vi "Example_Frames_To_Rows.vi"(8 "error in (no error)":errorcluster, 11 "frames":T1 {"flags" format="%.0x"; "id" format="%.0x"}) -> (0 "error out":errorcluster, 3 "rows":string[][](array[string]))   [LabVIEW 2021]
doc: "Example: formats the frames of one Read as table rows (time UTC s, ID hex, flags X/F/B/R/A/E, DLC, data hex) using Frame_Get. Allocates strings; for display only, not for a time-critical loop."
uses:
  api/CANsub_Channel/CANsub_Channel.lvclass
  <vilib>/JDP Science/JDP Science Common Utilities/JDP Utility.lvlib
  api/Typedefs/CANsub_Frames.ctl
  api/CANsub_API.lvlib
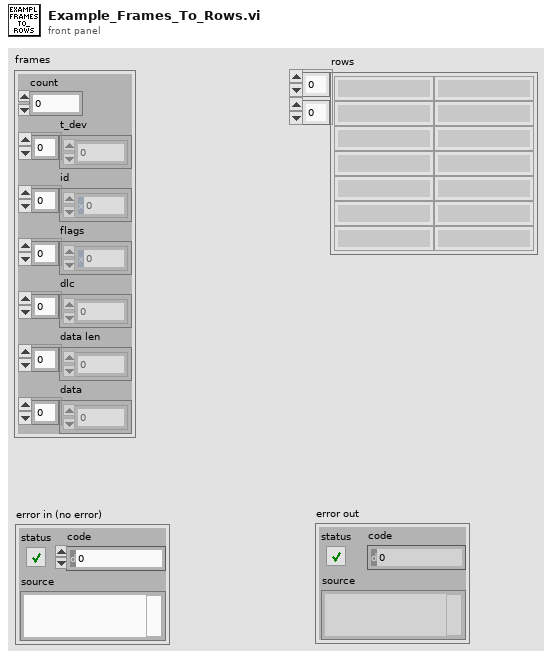
[diagram p1: front panel]
types:
  T1 = typedef "CANsub_API.lvlib/CANsub_Frames.ctl" = cluster{"count":i32, "t_dev":dbl[], "id":u32[], "flags":u16[], "dlc":u8[], "data len":u8[], "data":u8[]}
  T2 = typedef "CANsub_API.lvlib/CANsub_Frame.ctl" = cluster{"id":u32, "t_dev":dbl, "dlc":u8, "data len":u8, "ide":bool, "fdf":bool, "rtr":bool, "brs":bool, "esi":bool, "tx ack":bool, "error frame":bool}
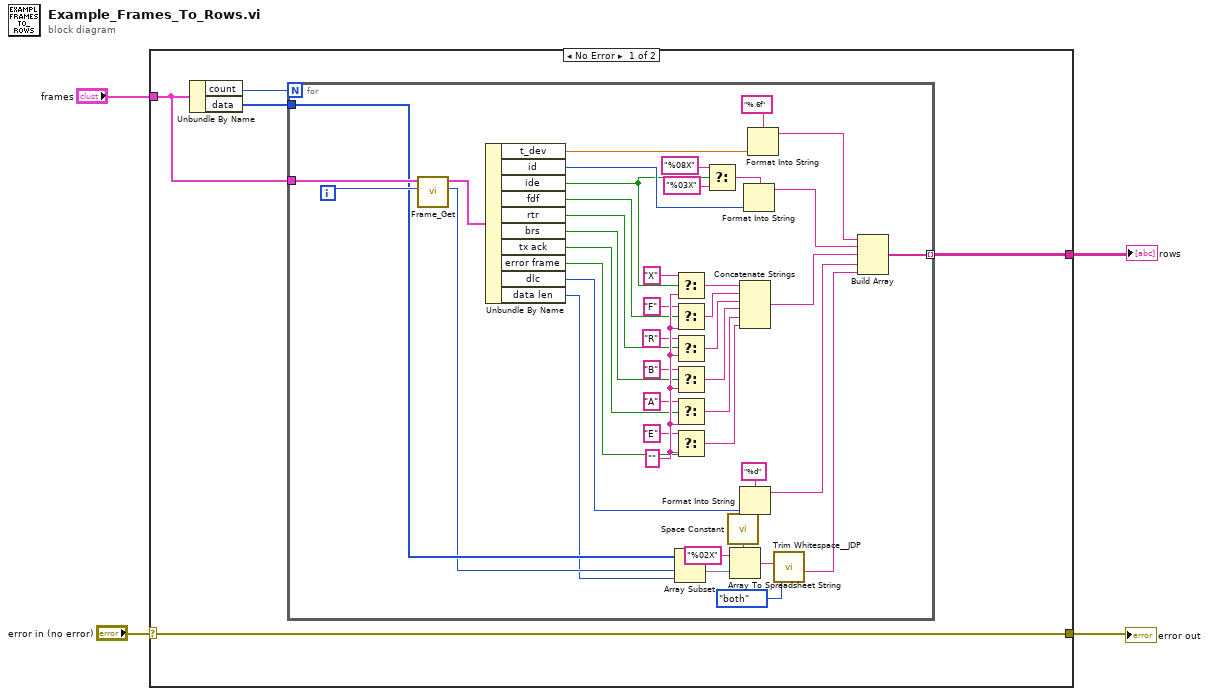
[diagram p0: block diagram]
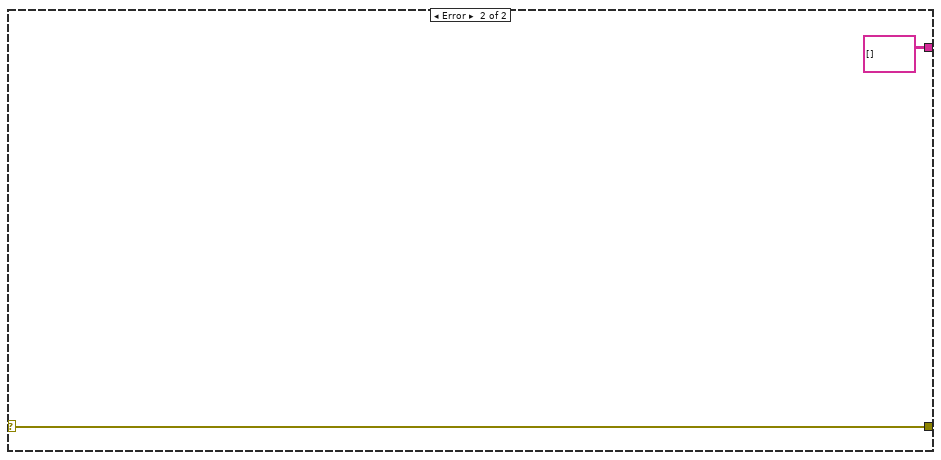
[diagram p2: hidden frame]
diagram:
  n1 = case shown="No Error" "error in (no error)" {
    selector: "error in (no error)" -> [w5 w54]
    tunnel: "frames" -> [w8 _]
    tunnel: [w6 string[][] []] -> w3
    tunnel: [w5 w54] -> w1
    frame No Error {
      n2 = Unbundle By Name(w8) -> ("count"=w9:i32, "data"=w7:u8[])
      n3 = for {
        N: w9 -> [_]
        tunnel: w8 -> [w53]
        tunnel: w7 -> [w23]
        tunnel: [w11] -> w6 mode=indexing
        i -> [w52]
        w47 = ""
        n4 = call "Frame_Get.vi"("i"=w52, "frames"=w53) -> ("data offset"=w22:i32, "frame"=w51:T2)  [unwired: 7 in, 1 out]
        n5 = Unbundle By Name(w51) -> ("t_dev"=w49:dbl, "id"=w48:u32, "ide"=w27:bool, "fdf"=w34:bool, "rtr"=w33:bool, "brs"=w32:bool, "tx ack"=w31:bool, "error frame"=w30:bool, "dlc"=w24:u8, "data len"=w21:u8)
        n6 = Array Subset(array=w23, index=w22, length=w21) -> (w18:u8[])
        n7 = Select(t="X", s=w27, f=w47) -> (s? t:f=w40:string)
        n8 = Select(t="F", s=w34, f=w47) -> (s? t:f=w39:string)
        n9 = Select(t="R", s=w33, f=w47) -> (s? t:f=w38:string)
        n10 = Select(t="B", s=w32, f=w47) -> (s? t:f=w37:string)
        n11 = Select(t="A", s=w31, f=w47) -> (s? t:f=w36:string)
        n12 = Select(t="E", s=w30, f=w47) -> (s? t:f=w35:string)
        n13 = Select(t="%08X" ("format string"), s=w27, f="%03X" ("format string")) -> (s? t:f=w26:string)
        n14 = call <vilib>:"Space Constant.vi"() -> ("String"=w20:string)
        n15 = Array To Spreadsheet String(delimiter (Tab)=w20, array=w18, 3:"%02X" ("format string")) -> (spreadsheet string=w17:string)
        n16 = Concatenate Strings(w40, w39, w38, w37, w36, w35) -> (w14:string)
        n17 = Format Into String(format string="%d", w24) -> (resulting string=w13:string)  [unwired: 2 in, 1 out]
        n18 = Format Into String(format string=w26, w48) -> (resulting string=w15:string)  [unwired: 2 in, 1 out]
        n19 = Format Into String(format string="%.6f", w49) -> (resulting string=w16:string)  [unwired: 2 in, 1 out]
        n20 = call <vilib>:"Trim Whitespace__JDP.vi"("Remove (leading and trailing)"=enum16{"leading", "trailing", "both"}."both", "String in"=w17) -> ("String out"=w12:string)  [unwired: 5 in]
        n21 = Build Array(w16, w15, w14, w13, w12) -> (w11:string[])
      }
    }
    frame Error {
    }
  }
  "rows" <- w3
  "error out" <- w1
